vi "Ctor Device.vi"(8 "error in (no error)":errorcluster, 11 "Device in":refnum<class "Device.lvclass">) -> (0 "error out":errorcluster, 3 "Device out":refnum<class "Device.lvclass">)   [LabVIEW 2020, in "HAL.lvlib" / "Device.lvclass"]
doc: "Ctor = Constructor VI. This VI should be used to create any DVRs or other references needed for your device driver. If using traditional data flow LVOOP programming, this VI does not need to be overridden.\n\nIf overridden, this VI should not try to perform any configuration or connect to a device, just get the class instance ready to be configured."
uses:
  Device.lvclass
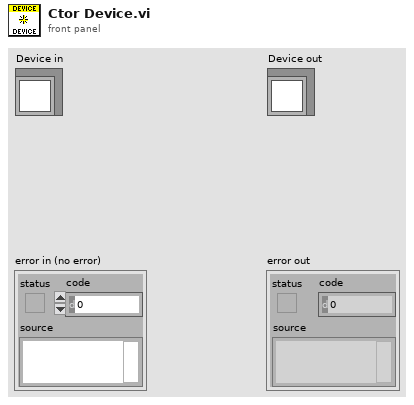
[diagram p1: front panel]
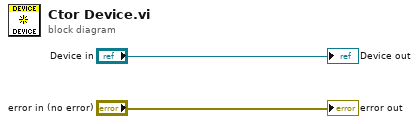
[diagram p0: block diagram]
diagram:
  "error out" <- "error in (no error)"
  "Device out" <- "Device in"
